vi "Set PWM Timing.vi"(6 "PWM Mode":T1, 7 "PWM Clock Divider":i32=1024, 8 "error in (no error)":errorcluster, 9 "Duty Cycle":dbl=0.5, 10 "PWM Freq":dbl=50.0, 11 "RPi PWM Pin in":T2=enum."GPIO12_PWM0_Pin32") -> (0 "error out":errorcluster, 1 "Actual Duty-Cycle":dbl, 2 "Actual Period":dbl=100.0, 3 "RPi PWM Pin out":T2=enum."GPIO12_PWM0_Pin32", 5 "PWM Timing":cluster{"PWM Range":u32, "PWM Data":u32})   [LabVIEW 2020, in "wiringPi.lvlib"]
doc: "<b>_______________________________________________________________</b>\n** Author: Juan José Villacorta\n** LabVIEW wrapper for C library <b> wiringPi </b>,\n** https://github.com/WiringPi/WiringPi\n<b>_______________________________________________________________</b>\n\nSet the PWM frequency and duty-cycle"
uses:
  wiringPi.lvlib
  <vilib>/ErrorRing/Error Ring.xnode
  Type Defs/PWM Mode.ctl
  Type Defs/GPIO Mode.ctl
  <vilib>/Utility/error.llb/Error Cluster From Error Code.vi
  Type Defs/GPIO Pins.ctl
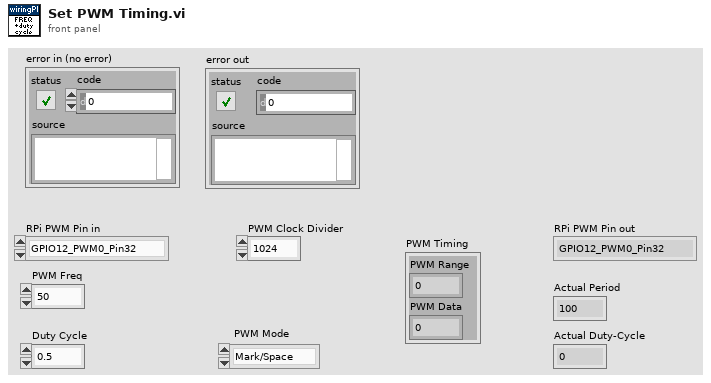
[diagram p1: front panel]
types:
  T1 = typedef "wiringPi.lvlib/PWM Mode.ctl" = enum16{"Mark/Space", "Balanced"}
  T2 = typedef "wiringPi.lvlib/GPIO Pins.ctl" = enum32{"GPIO0_I2C0_SDA_Pin27", "GPIO1_I2C0_SDA1_Pin28", "GPIO2_I2C1_SDA_Pin3", "GPIO3_I2C1_SCL_Pin5", "GPIO4_GPCLK0_Pin7", "GPIO5_GPCLK1_Pin29", "GPIO6_GPCLK2_Pin31", "GPIO7_SPI_CE1_N_Pin26", "GPIO8_SPI_CE0_N_Pin24", "GPIO9_SPI0_MISO_Pin21", "GPIO10_SPI0_MOSI_Pin19", "GPIO11_SPI0_CLK_Pin23", "GPIO12_PWM0_Pin32", "GPIO13_PWM1_Pin33", "GPIO14_TXD0_Pin8", "GPIO15_RXD0_Pin10", "GPIO16_Pin36", "GPIO17_Pin11", "GPIO18_PWM0_Pin12", "GPIO19_PWM1_Pin35", "GPIO20_GPCLK0_Pin38", "GPIO21_GPCLK1_Pin40", "GPIO22_Pin15", "GPIO23_Pin16", "GPIO24_Pin18", "GPIO25_Pin22", "GPIO26_Pin37", "GPIO27_Pin13"}
  T3 = typedef "wiringPi.lvlib/GPIO Mode.ctl" = u16
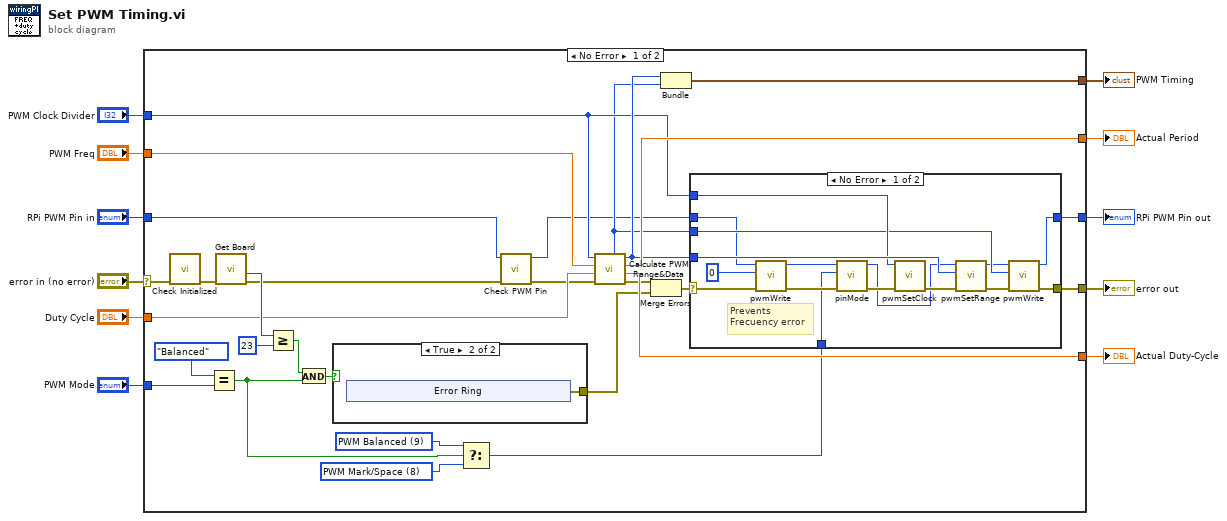
[diagram p0: block diagram]
diagram:
  n1 = case shown="No Error" "error in (no error)" {
    selector: "error in (no error)" -> [w15 w65]
    tunnel: [w40 w65] -> w11
    tunnel: "PWM Freq" -> [w39 _]
    tunnel: "RPi PWM Pin in" -> [w13 w66]
    tunnel: [w36 _] -> w8
    tunnel: "PWM Clock Divider" -> [w21 _]
    tunnel: [w35 _] -> w6
    tunnel: [w34 _] -> w5
    tunnel: "PWM Mode" -> [w25 _]
    tunnel: [w20 w66] -> w2
    tunnel: "Duty Cycle" -> [w18 _]
    frame No Error {
      w27 = T3 8 items=["Input"=0, "Output"=1, "PWM"=2, "PWM Mark/Space"=8, "PWM Balanced"=9, "Clock"=3, "Software PWM"=4, "Sofware Tono"=5, "PWM Tone"=6, "Off"=7] ("Mode")
      w26 = T3 9 items=["Input"=0, "Output"=1, "PWM"=2, "PWM Mark/Space"=8, "PWM Balanced"=9, "Clock"=3, "Software PWM"=4, "Sofware Tono"=5, "PWM Tone"=6, "Off"=7] ("Mode")
      n2 = call "Check Initialized.vi"("error in (no error)"=w15) -> ("error out"=w14:errorcluster)  [unwired: 10 in]
      n3 = Equal?(x=PWM_Mode."Balanced" ("y"), y=w25) -> (x = y?=w24:bool)
      n4 = call "Get Board.vi"("error in (no error)"=w14) -> ("error out"=w17:errorcluster, "Model Number"=w38:i32)  [unwired: 7 in, 2 out]
      n5 = Greater Or Equal?(x=w38, y=23) -> (x >= y?=w33:bool)
      n6 = And(x=w33, y=w24) -> (x .and. y?=w32:bool)
      n7 = case shown="True" w32 {
        tunnel: [_ w41] -> w30
        frame False {
        }
        frame True {
          n8 = xnode "Error Ring"() -> ("error out"=w41:errorcluster)
        }
      }
      n9 = Select(t=w26, s=w24, f=w27) -> (s? t:f=w23:T3)
      n10 = call "Check PWM Pin.vi"("error in (no error)"=w17, "RPi PWM Pin in"=w13) -> ("error out"=w16:errorcluster, "RPi PWM Pin out"=w12:T2)  [unwired: 8 in]
      n11 = call "Calculate PWM Range&Data.vi"("error in (no error)"=w16, "Duty Cycle"=w18, "PWM Freq"=w39, "PWM Clock Divider"=w21) -> ("error out"=w31:errorcluster, "Actual Duty Cycle"=w35:dbl, "Actual Freq"=w36:dbl, "PWM Range"=w22:i32, "PWM Data"=w19:i32)  [unwired: 3 in]
      n12 = Merge Errors(w31, w30) -> (w29:errorcluster)
      n13 = Bundle("PWM Range"=w22, "PWM Data"=w19) -> (w34:cluster{"PWM Range":i32, "PWM Data":i32})  [unwired: 1 in]
      n14 = case shown="No Error" w29 {
        selector: w29 -> [w62 w64]
        tunnel: [w52 w64] -> w40
        tunnel: w12 -> [w49 w63]
        tunnel: w23 -> [w59 _]
        tunnel: w22 -> [w57 _]
        tunnel: w21 -> [w56 _]
        tunnel: [w51 w63] -> w20
        tunnel: w19 -> [w50 _]
        frame No Error {
          # "Prevents\nFrecuency error"
          n15 = call "pwmWrite.vi"("error in (no error)"=w62, "Value"=0, "RPi Pin"=w49) -> ("error out"=w60:errorcluster, "RPi Pin out"=w58:T2)  [unwired: 7 in]
          n16 = call "pinMode.vi"("error in (no error)"=w60, "Mode"=w59, "RPi Pin"=w58) -> ("error out"=w55:errorcluster, "RPi Pin out"=w47:T2)  [unwired: 7 in]
          n17 = call "pwmSetClock.vi"("error in (no error)"=w55, "Divisor"=w56) -> ("error out"=w54:errorcluster)  [unwired: 9 in]
          n18 = call "pwmSetRange.vi"("error in (no error)"=w54, "Value"=w57, "RPi Pin"=w47) -> ("error out"=w53:errorcluster, "RPi Pin out"=w48:T2)  [unwired: 7 in]
          n19 = call "pwmWrite.vi"("error in (no error)"=w53, "Value"=w50, "RPi Pin"=w48) -> ("error out"=w52:errorcluster, "RPi Pin out"=w51:T2)  [unwired: 7 in]
        }
        frame Error {
        }
      }
    }
    frame Error {
    }
  }
  "error out" <- w11
  "RPi PWM Pin out" <- w2
  "Actual Period" <- w8
  "Actual Duty-Cycle" <- w6
  "PWM Timing" <- w5
